vi "FuncVI-FileListDir.vi"(5 "InstanceRef":T2, 9 "arg list":T1[](array[typedef]) {"num" format="%.2f"}) -> (0 "error out":bool, 3 "result":T1 {"num" format="%.2f"})   [LabVIEW 2021]
doc: "::: CalcExpress Toolkit :::\nCopyright (c) 2000-2026 Konstantin Shifershteyn. All rights reserved."
uses:
  cetypes.llb/CalcExpress Function Argument Info.ctl
  cetypes.llb/CalcExpress Instance RefNum.ctl
panel:
  in  "max arg num":i32=3
  in  "min arg num":i32=1
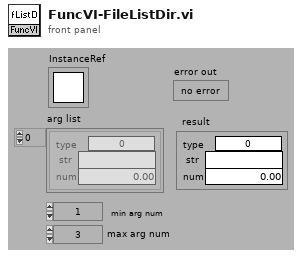
[diagram p1: front panel]
types:
  T1 = typedef "CalcExpress Function Argument Info.ctl" = cluster{"type":u32, "str":string, "num":dbl}
  T2 = typedef "CalcExpress Instance RefNum.ctl" = refnum<k1>
  T3 = cluster{"index":i32, "data type":enum32{"String", "DBL Number", "identifier", "1D Array of DBL", "2D Array of DBL", "CDB Number", "1D Array of CDB", "2D Array of CDB", "1D Array of String", "2D Array of String", "Unknown data type"}, "default num":dbl, "default str":string}[]
  T4 = enum32{"String", "DBL Number", "identifier", "1D Array of DBL", "2D Array of DBL", "CDB Number", "1D Array of CDB", "2D Array of CDB", "1D Array of String", "2D Array of String", "Unknown data type"}
  T5 = enum32{"existing file", "new file", "new or existing file", "existing dir", "new dir", "new or existing dir", "existing file (use LLBs)", "new file (use LLBs)", "new or existing file (use LLBs)", "new or existing file or directory (use LLBs)", "existing dir (use LLBs)", "new dir (use LLBs)", "new or existing dir (use LLBs)", "existing file or dir", "new file or dir", "new or existing file or dir", "existing file or dir (use LLBs)", "new file or dir (use LLBs)"}
  T6 = cluster{"type: use this constant to specify a predefined type code":enum32{"String", "DBL Number", "identifier", "1D Array of DBL", "2D Array of DBL", "CDB Number", "1D Array of CDB", "2D Array of CDB", "1D Array of String", "2D Array of String", "Unknown data type"}, "data string":string, dbl}
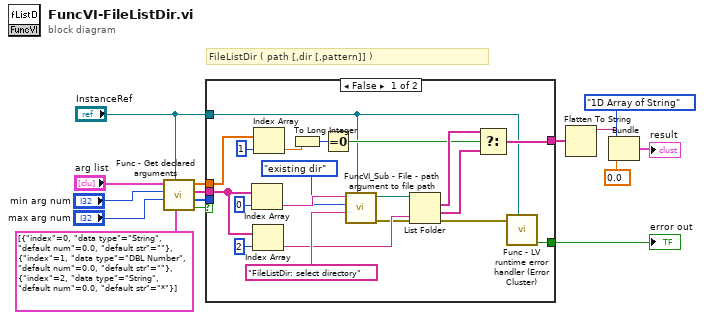
[diagram p0: block diagram]
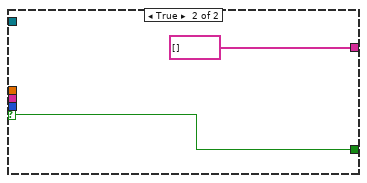
[diagram p2: hidden frame]
diagram:
  # "FileListDir ( path [,dir [,pattern]] )"
  n1 = call "Func - Get declared arguments.vi"("arg descriptors"=T3 [{"index"=0, "data type"=enum."String", "default num"=0.0, "default str"=""}, {"index"=1, "data type"=enum."DBL Number", "default num"=0.0, "default str"=""}, {"index"=2, "data type"=enum."String", "default num"=0.0, "default str"="*"}] ("args descriptors"), "InstanceRef"="InstanceRef", "max arg num"="max arg num", "min arg num"="min arg num", "arg list"="arg list") -> ("error out"=w9:bool, "type list"=w7:u32[], "str list"=w10:string[], "num list"=w8:dbl[])  [unwired: 3 in]
  n2 = case shown="False" w9 {
    selector: w9 -> [_ w37]
    tunnel: [w16 w37] -> w13
    tunnel: "InstanceRef" -> [w17 _]
    tunnel: w10 -> [w33 _]
    tunnel: w8 -> [w23 _]
    tunnel: w7 -> [_ _]
    tunnel: [w19 string[] []] -> w3
    frame False {
      n3 = Index Array(array=w33, index=0) -> (element=w32:string)
      n4 = Index Array(array=w33, index=2) -> (element=w28:string)
      n5 = Index Array(array=w23, index=1) -> (element=w22:dbl)
      n6 = To Long Integer(number=w22) -> (32bit integer=w21:i32)
      n7 = Equal To 0?(x=w21) -> (x = 0?=w20:bool)
      n8 = call "FuncVI_Sub - File - path argument to file path.vi"("InstanceRef"=w17, "prompt"="FileListDir: select directory", "select mode (2)"=T5."existing dir", "arg: file path"=w32) -> ("error out"=w27:errorcluster, "file path"=w29:path)  [unwired: 5 in, 1 out]
      n9 = List Folder(path=w29, pattern=w28, error in=w27) -> (filenames=w26:string[], folder names=w25:string[], error out=w18:errorcluster)  [unwired: 1 in, 1 out]
      n10 = Select(t=w26, s=w20, f=w25) -> (s? t:f=w19:string[])
      n11 = call "Func - LV runtime error handler (Error Cluster).vi"("InstanceRef"=w17, "LabVIEW error"=w18) -> ("error out"=w16:bool)  [unwired: 4 in, 3 out]
    }
    frame True {
    }
  }
  "error out" <- w13
  n12 = Flatten To String(anything=w3) -> (data string=w4:string)  [unwired: 3 in, 2 out]
  n13 = Bundle("type: use this constant to specify a predefined type code"=T4."1D Array of String", "data string"=w4, 0.0) -> (→"result":T6)  [unwired: 1 in]
